vi "Supervisor_Shutdown_Procedure.vi"(8 "error in (no error)":errorcluster={"status"=FALSE, "code"=0, "source"="\"\""}, 10 "shutdown reason":string, 11 "TestDefinition":string) -> (0 "error out":errorcluster={"status"=FALSE, "code"=0, "source"="\"\""}, 2 "status ok":bool, 3 "Completion/timeout":string)   [LabVIEW 2026]
doc: "INTENT: Execute exactly one test-specific shutdown sequence. LOGIC: Run bounded approved shutdown actions if safe; when unavailable rely on protective fallback and record outcome."
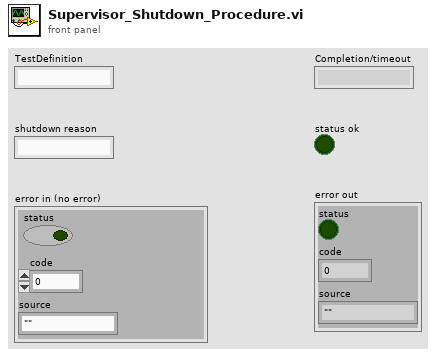
[diagram p1: front panel]
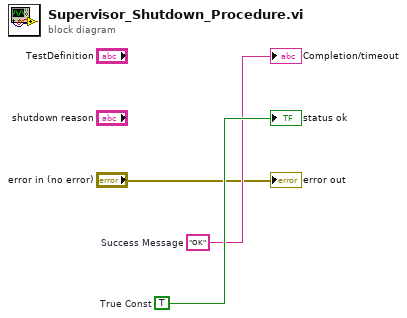
[diagram p0: block diagram]
diagram:
  w3 = TRUE  # True Const
  w2 = "OK"  # Success Message
  "Completion/timeout" <- w2
  "status ok" <- w3
  "error out" <- "error in (no error)"
